vi "T-Set_Change.vi"(11 "T set":string="5E3") -> ()   [LabVIEW 2024]
uses:
  GPIB_Address.vi
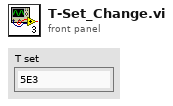
[diagram p1: front panel]
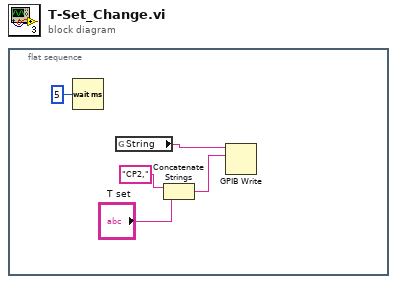
[diagram p0: block diagram]
diagram:
  n1 = flat-sequence {
    frame #0 {
      n2 = Wait (ms)(milliseconds to wait=u32 5) -> ()  [unwired: 1 out]
      n3 = global read "GPIB_Address.vi" "String"() -> (w5:string)
      n4 = Concatenate Strings("CP2," ("string"), "T set") -> (w2:string)
      n5 = GPIB Write(0:w5, 1:w2) -> ()  [unwired: 3 in, 2 out]
    }
  }
